vi "Sous_VI_recule.vi"(8 "error in (no error)":errorcluster) -> (0 "error out":errorcluster)   [LabVIEW 2017]
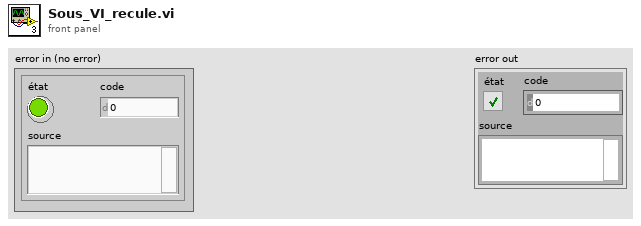
[diagram p1: front panel]
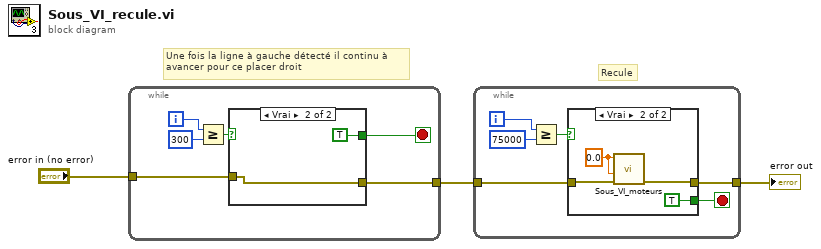
[diagram p0: block diagram]
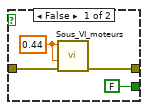
[diagram p2: hidden frame]
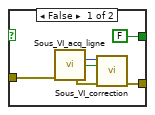
[diagram p3: hidden frame]
diagram:
  # "Recule"
  # "Une fois la ligne à gauche détecté il continu à \navancer pour ce placer droit"
  n1 = while {
    tunnel: "error in (no error)" -> [w5]
    tunnel: [w4] -> w2
    i -> [w6]
    stop <- w8 stop-if-true
    n2 = Greater Or Equal?(x=w6, y=300) -> (x >= y?=w9:bool)
    n3 = case shown="Vrai" w9 {
      tunnel: [FALSE TRUE] -> w8
      tunnel: w5 -> [w12 w16]
      tunnel: [w10 w16] -> w4
      frame False {
        n4 = call "Sous_VI_acq_ligne.vi"("error in (no error)"=w12) -> ("Décalage"=w14:u32, "G/D ?"=w13:bool, "error out"=w11:errorcluster)  [unwired: 9 in, 3 out]
        n5 = call "Sous_VI_correction.vi"("error in (no error)"=w11, "G/D ?"=w13, "Décalage"=w14) -> ("error out"=w10:errorcluster)  [unwired: 8 in]
      }
      frame True {
      }
    }
  }
  n6 = while {
    tunnel: w2 -> [w19]
    tunnel: [w18] -> w1
    i -> [w20]
    stop <- w22 stop-if-true
    n7 = Greater Or Equal?(x=w20, y=75000) -> (x >= y?=w23:bool)
    n8 = case shown="Vrai" w23 {
      tunnel: [FALSE TRUE] -> w22
      tunnel: w19 -> [w25 w29]
      tunnel: [w24 w28] -> w18
      frame False {
        w26 = 0.44 ("moteur gauche vite")
        n9 = call "Sous_VI_moteurs.vi"("error in (no error)"=w25, "Moteur Droit"=w26, "Moteur Gauche"=w26) -> ("error out"=w24:errorcluster)  [unwired: 8 in]
      }
      frame True {
        w30 = 0.0 ("Moteur Gauche")
        n10 = call "Sous_VI_moteurs.vi"("error in (no error)"=w29, "Moteur Droit"=w30, "Moteur Gauche"=w30) -> ("error out"=w28:errorcluster)  [unwired: 8 in]
      }
    }
  }
  "error out" <- w1
